vi "Set CO3000 Reference.vi"(8 "error in (no error)":errorcluster caption="에러 입력(에러 없음)", 11 "Instrument Manager 입력":refnum<class "Instrument Manager.lvclass">) -> (0 "error out":errorcluster caption="에러 출력", 3 "Instrument Manager 출력":refnum<class "Instrument Manager.lvclass">)   [LabVIEW 2023, in "Instrument Manager.lvclass"]
uses:
  Instrument Manager.lvclass
  Instrument Manager.lvclass/Instrument Manager.ctl
  0aa25dca-f31f-4714-bd46-85d206e1e70f.vi
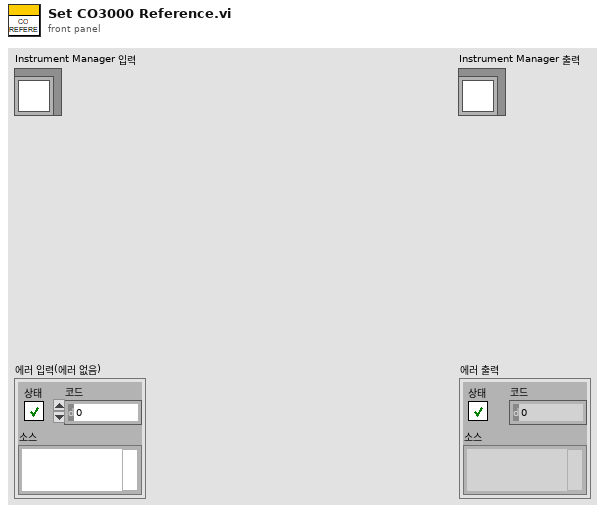
[diagram p1: front panel]
types:
  T1 = cluster{"Target Angle":dbl, "Turn Table Speed":i32, "Fetch Interval":i32}
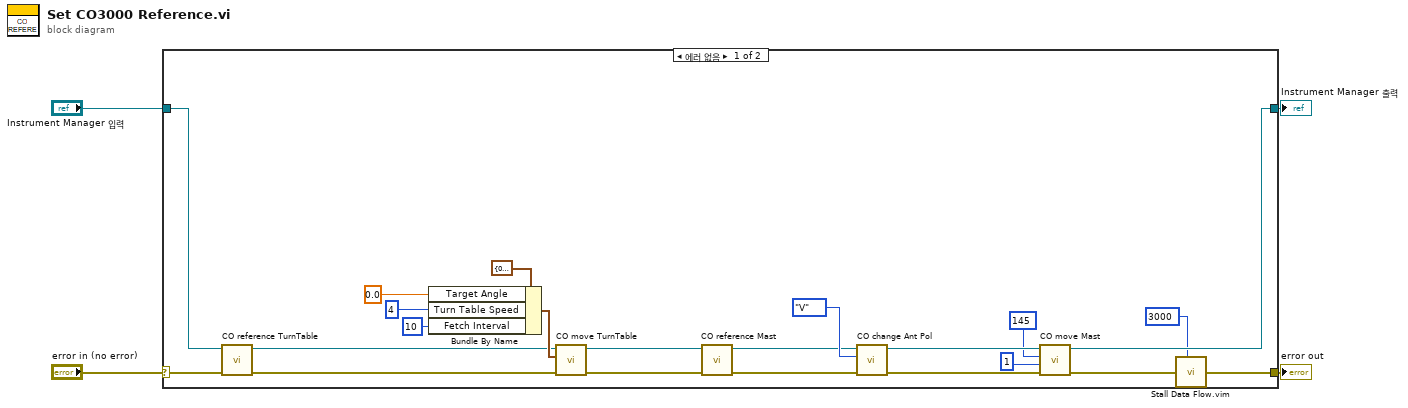
[diagram p0: block diagram]
diagram:
  n1 = case shown="에러 없음" "error in (no error)" {
    selector: "error in (no error)" -> [w22 w28]
    tunnel: [w6 w28] -> w3
    tunnel: [w12 w27] -> w1
    tunnel: "Instrument Manager 입력" -> [w17 w27]
    frame No Error {
      n2 = call "CO reference TurnTable.vi"("error in (no error)"=w22, "Instrument Manager 입력"=w17) -> ("error out"=w11:errorcluster, "Instrument Manager 출력"=w8:refnum<class "Instrument Manager.lvclass">)  [unwired: 8 in]
      n3 = Bundle By Name(cluster=T1 {"Target Angle"=0.0, "Turn Table Speed"=0, "Fetch Interval"=0} ("Turn Table Info"), "Target Angle"=0.0, "Turn Table Speed"=4, "Fetch Interval"=10) -> (w18:T1)
      n4 = call "CO move TurnTable.vi"("error in (no error)"=w11, "Turn Table Info"=w18, "Instrument Manager 입력"=w8) -> ("error out"=w10:errorcluster, "Instrument Manager 출력"=w9:refnum<class "Instrument Manager.lvclass">)  [unwired: 7 in]
      n5 = call "CO reference Mast.vi"("error in (no error)"=w10, "Instrument Manager 입력"=w9) -> ("error out"=w20:errorcluster, "Instrument Manager 출력"=w19:refnum<class "Instrument Manager.lvclass">)  [unwired: 8 in]
      n6 = call "CO change Ant Pol.vi"("error in (no error)"=w20, "Antenna Pol"=enum16{"H", "V"}."V", "Instrument Manager 입력"=w19) -> ("error out"=w16:errorcluster, "Instrument Manager 출력"=w15:refnum<class "Instrument Manager.lvclass">)  [unwired: 7 in]
      n7 = call "CO move Mast.vi"("error in (no error)"=w16, "Speed (1~8)"=1, "Height (100~400)"=145, "Instrument Manager 입력"=w15) -> ("error out"=w7:errorcluster, "Instrument Manager 출력"=w12:refnum<class "Instrument Manager.lvclass">)  [unwired: 6 in]
      n8 = call "Stall Data Flow.vim"("value in"=w7, "milliseconds to wait"=u32 3000) -> ("value out"=w6:errorcluster)  [unwired: 1 out]
    }
    frame Error {
    }
  }
  "error out" <- w3
  "Instrument Manager 출력" <- w1
